vi "Controller.vi"(8 "error in":errorcluster, 9 "TimeNow":dbl, 10 "Command":T4, 11 "InData":T1) -> (0 "error out":errorcluster, 3 "OutData":T1)   [LabVIEW 2026]
uses:
  Controls/DataType.ctl
  Controls/StateType.ctl
  Controls/ModeType.ctl
  Controls/CommandType.ctl
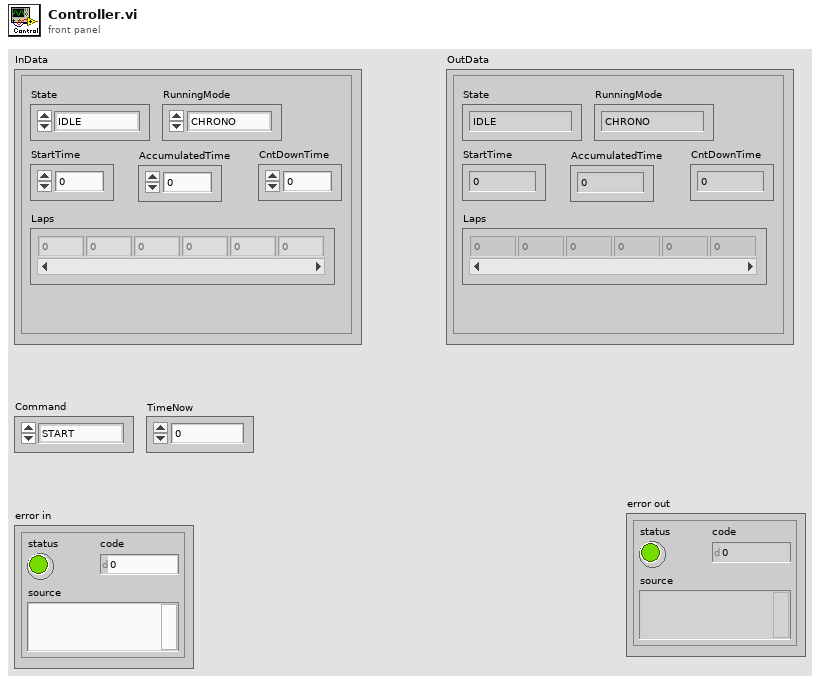
[diagram p1: front panel]
types:
  T1 = typedef "DataType.ctl" = cluster{"State":T2, "RunningMode":T3, "StartTime":dbl, "AccumulatedTime":dbl, "CntDownTime":dbl, "Laps":dbl[]}
  T2 = typedef "StateType.ctl" = enum16{"IDLE", "RUNNING", "PAUSED", "FINISHED"}
  T3 = typedef "ModeType.ctl" = enum16{"CHRONO", "COUNTDOWN", ""}
  T4 = typedef "CommandType.ctl" = enum16{"START", "STOP", "RESET", "LAP", "MODE", "TICK"}
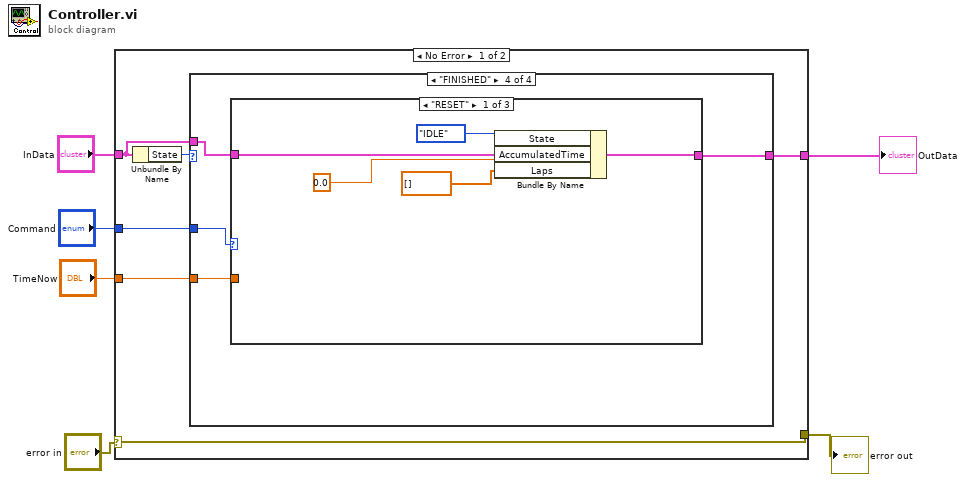
[diagram p0: block diagram]
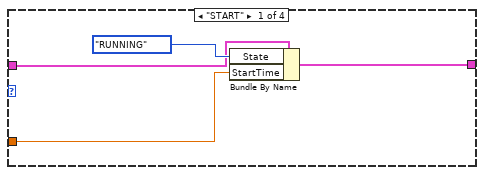
[diagram p3: hidden frame]
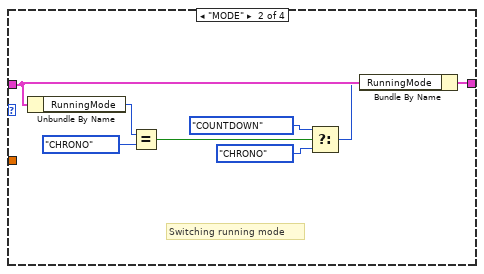
[diagram p4: hidden frame]
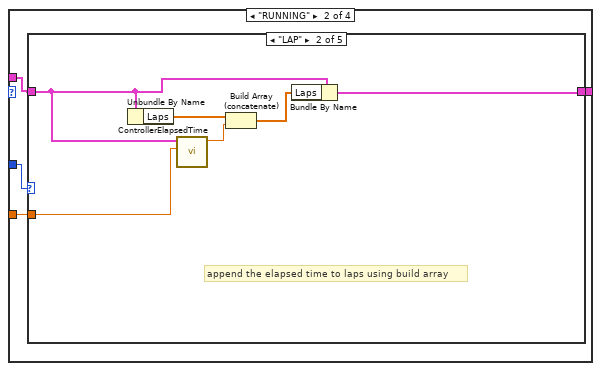
[diagram p6: hidden frame]
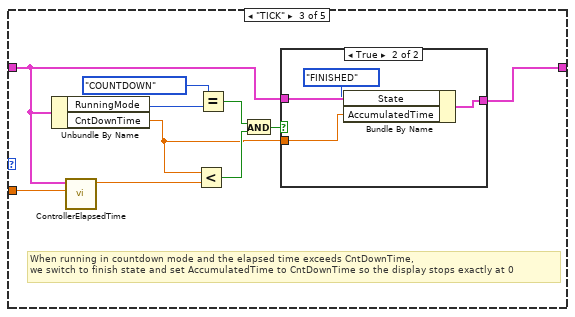
[diagram p8: hidden frame]
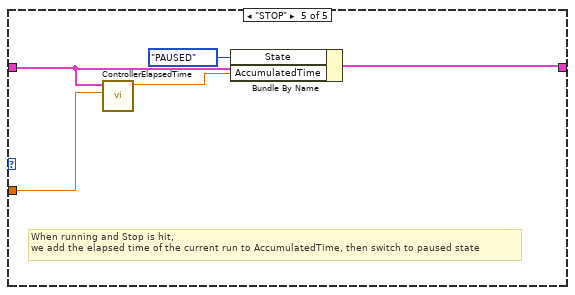
[diagram p11: hidden frame]
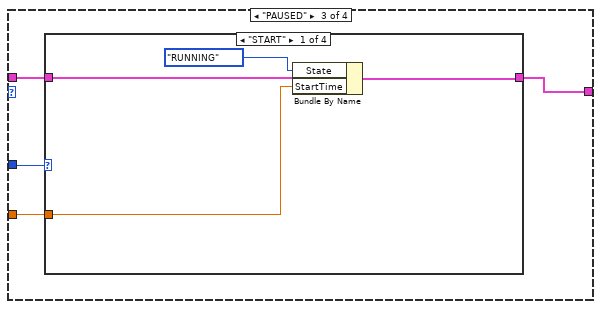
[diagram p12: hidden frame]
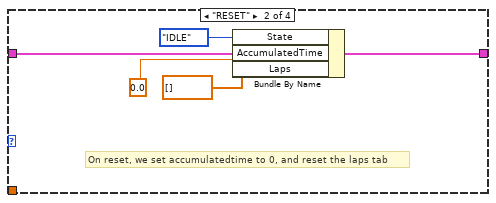
[diagram p13: hidden frame]
diagram:
  n1 = case shown="No Error" "error in" {
    selector: "error in" -> [w12 w90]
    tunnel: [w12 w90] -> w5
    tunnel: "InData" -> [w8 w89]
    tunnel: [w9 w89] -> w3
    tunnel: "Command" -> [w10 _]
    tunnel: "TimeNow" -> [w7 _]
    frame No Error {
      n2 = Unbundle By Name(w8) -> ("State"=w11:T2)
      n3 = case shown="\"FINISHED\"" w11 {
        tunnel: w10 -> [w16 w34 w64 w81]
        tunnel: [w13 w33 w66 w80] -> w9
        tunnel: w8 -> [w15 w32 w65 w79]
        tunnel: w7 -> [w14 w31 w63 w78]
        frame "IDLE" {
          n4 = case shown="\"STOP\"" w16 {
            tunnel: w15 -> [w18 w28 w29 w30]
            tunnel: w14 -> [w19 _ _ _]
            tunnel: [w17 w21 w29 w30] -> w13
            frame "START" {
              n5 = Bundle By Name(cluster=w18, "State"=StateType."RUNNING", "StartTime"=w19) -> (w17:T1)
            }
            frame "MODE" {
              # "Switching running mode"
              n6 = Unbundle By Name(w28) -> ("RunningMode"=w27:T3)
              n7 = Equal?(x=w27, y=ModeType."CHRONO") -> (x = y?=w25:bool)
              n8 = Select(t=ModeType."COUNTDOWN", s=w25, f=ModeType."CHRONO" ("y")) -> (s? t:f=w24:T3)
              n9 = Bundle By Name(cluster=w28, "RunningMode"=w24) -> (w21:T1)
            }
            frame Default {
            }
            frame "STOP" {
            }
          }
        }
        frame "RUNNING" {
          n10 = case shown="\"LAP\"" w34 {
            tunnel: w32 -> [w35 w37 w43 w57 w61]
            tunnel: [w35 w36 w44 w57 w58] -> w33
            tunnel: w31 -> [_ w41 w51 _ w60]
            frame "START" {
            }
            frame "LAP" {
              # "append the elapsed time to laps using build array"
              n11 = Unbundle By Name(w37) -> ("Laps"=w40:dbl[])
              n12 = call "ControllerElapsedTime.vi"("TimeNow"=w41, "InData"=w37) -> ("Elapsed"=w39:dbl)  [unwired: 9 in]
              n13 = Build Array (concatenate)(w40, w39) -> (w38:dbl[])
              n14 = Bundle By Name(cluster=w37, "Laps"=w38) -> (w36:T1)
            }
            frame "TICK" {
              # "When running in countdown mode and the elapsed time exceeds CntDownTime,\nwe switch to finish state and set AccumulatedTime to CntDownTime so the display stops exactly at 0"
              n15 = Unbundle By Name(w43) -> ("RunningMode"=w49:T3, "CntDownTime"=w42:dbl)
              n16 = call "ControllerElapsedTime.vi"("TimeNow"=w51, "InData"=w43) -> ("Elapsed"=w50:dbl)  [unwired: 9 in]
              n17 = Less?(x=w42, y=w50) -> (x < y?=w46:bool)
              n18 = Equal?(x=ModeType."COUNTDOWN", y=w49) -> (x = y?=w47:bool)
              n19 = And(x=w47, y=w46) -> (x .and. y?=w45:bool)
              n20 = case shown="True" w45 {
                tunnel: w43 -> [w52 w56]
                tunnel: [w52 w55] -> w44
                tunnel: w42 -> [_ w53]
                frame False {
                }
                frame True {
                  n21 = Bundle By Name(cluster=w56, "State"=StateType."FINISHED", "AccumulatedTime"=w53) -> (w55:T1)
                }
              }
            }
            frame Default {
            }
            frame "STOP" {
              # "When running and Stop is hit,\nwe add the elapsed time of the current run to AccumulatedTime, then switch to paused state"
              n22 = call "ControllerElapsedTime.vi"("TimeNow"=w60, "InData"=w61) -> ("Elapsed"=w59:dbl)  [unwired: 9 in]
              n23 = Bundle By Name(cluster=w61, "State"=StateType."PAUSED", "AccumulatedTime"=w59) -> (w58:T1)
            }
          }
        }
        frame "PAUSED" {
          n24 = case shown="\"START\"" w64 {
            tunnel: [w68 w71 w76 w77] -> w66
            tunnel: w65 -> [w67 w74 w76 w77]
            tunnel: w63 -> [w69 _ _ _]
            frame "START" {
              n25 = Bundle By Name(cluster=w67, "State"=StateType."RUNNING", "StartTime"=w69) -> (w68:T1)
            }
            frame "RESET" {
              # "On reset, we set accumulatedtime to 0, and reset the laps tab"
              n26 = Bundle By Name(cluster=w74, "State"=StateType."IDLE", "AccumulatedTime"=0.0 ("StartTime"), "Laps"=dbl[] []) -> (w71:T1)
            }
            frame Default {
            }
            frame "STOP" {
            }
          }
        }
        frame "FINISHED" {
          n27 = case shown="\"RESET\"" w81 {
            tunnel: [w85 w87 w88] -> w80
            tunnel: w79 -> [w86 w87 w88]
            tunnel: w78 -> [_ _ _]
            frame "RESET" {
              n28 = Bundle By Name(cluster=w86, "State"=StateType."IDLE", "AccumulatedTime"=0.0, "Laps"=dbl[] []) -> (w85:T1)
            }
            frame Default {
            }
            frame "STOP" {
            }
          }
        }
      }
    }
    frame Error {
    }
  }
  "error out" <- w5
  "OutData" <- w3
